vi "Test Report Generation.vi"(8 "error in (no error)":errorcluster) -> (0 "error out":errorcluster, 3 "Succeeded?":bool)   [LabVIEW 2020]
uses:
  classes/Test Suite/Define Test Suite (SimpleText Report).vi
  classes/Test Suite/Test Suite.lvclass
panel:
  out "Test Report File Contents":string
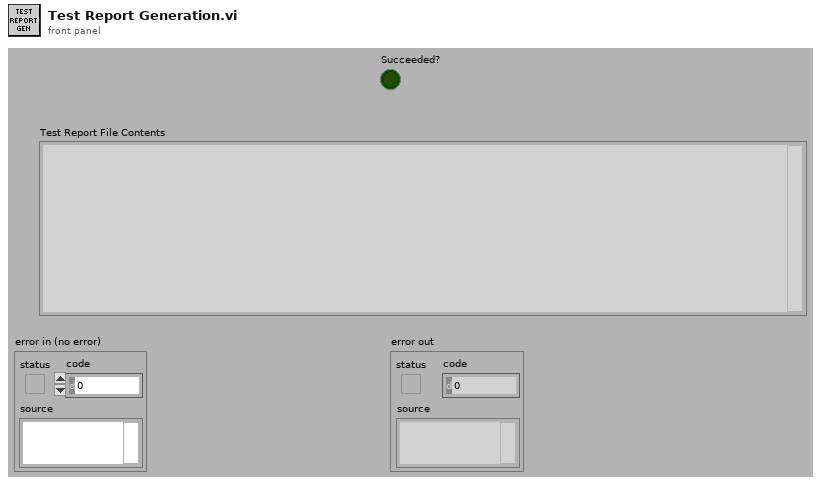
[diagram p1: front panel]
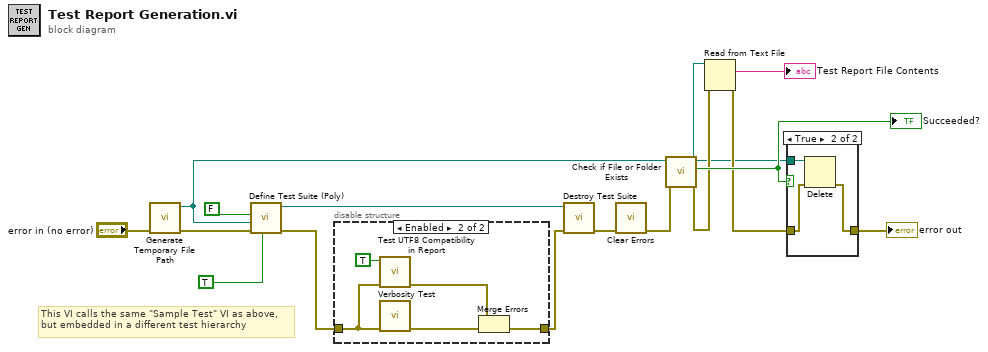
[diagram p0: block diagram]
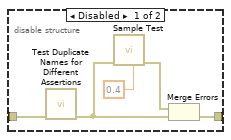
[diagram p2: hidden frame]
diagram:
  # "This VI calls the same \"Sample Test\" VI as above,\nbut embedded in a different test hierarchy"
  n1 = call <vilib>:"Generate Temporary File Path.vi"("error in (no error)"="error in (no error)") -> ("error out"=w7:errorcluster, "Unique Temporary File Path"=w6:path)  [unwired: 9 in]
  n2 = call-poly "Define Test Suite (Poly).vi"("Verbose (F)"=TRUE, "error in (no error)"=w7, "Report Path"=w6, "Interactive"=FALSE) -> ("error out"=w4:errorcluster, "Test Suite"=w8:refnum<class "Test Suite.lvclass">)  [unwired: 5 in, 1 out]
  n3 = disable-structure shown="Enabled" {
    disable-tunnel: [w21 w23] -> w5
    disable-tunnel: w4 -> [w19 w26]
    frame Disabled {
      n4 = call "Test Duplicate Names for Different Assertions.vi"("error in (no error)"=w19) -> ("error out"=w18:errorcluster)  [unwired: 10 in]
      n5 = call "Sample Test.vi"("Execution time (s)"=0.4, "error in (no error)"=w18) -> ("error out"=w20:errorcluster)  [unwired: 9 in]
      n6 = Merge Errors(w20, w18) -> (w21:errorcluster)
    }
    frame Enabled {
      n7 = call "Test UTF8 Compatibility in Report.vi"("error in (no error)"=w26, "Force FAIL?"=TRUE) -> ("error out"=w24:errorcluster)  [unwired: 9 in]
      n8 = call "Verbosity Test.vi"("error in (no error)"=w26) -> ("error out"=w25:errorcluster)  [unwired: 10 in]
      n9 = Merge Errors(w24, w25) -> (w23:errorcluster)
    }
  }
  n10 = call-dynamic "Destroy Test Suite.vi"("error in (no error)"=w5, "Test Suite in"=w8) -> ("error out"=w2:errorcluster)  [unwired: 8 in, 1 out]
  n11 = call <vilib>:"Clear Errors.vi"("error in (no error)"=w2) -> ("error out"=w1:errorcluster)  [unwired: 5 in, 1 out]
  n12 = call <vilib>:"Check if File or Folder Exists.vi"("error in (no error)"=w1, "path"=w6) -> ("error out"=w13:errorcluster, "file or folder exists?"=w15:bool, "dup path"=w10:path)  [unwired: 7 in]
  "Succeeded?" <- w15
  n13 = Read from Text File(file (use dialog)=w10, error in=w13) -> (text=→"Test Report File Contents":string, error out=w12:errorcluster)  [unwired: 2 in, 2 out]
  n14 = case shown="True" w15 {
    tunnel: w10 -> [_ w30]
    tunnel: w12 -> [w27 w29]
    tunnel: [w27 w28] -> w14
    frame False {
    }
    frame True {
      n15 = Delete(path (use dialog)=w30, error in=w29) -> (error out=w28:errorcluster)  [unwired: 3 in, 2 out]
    }
  }
  "error out" <- w14
